vi "Main.vi"() -> ()   [LabVIEW 2017]
doc: "The myRIO Project template acquires acceleration data from the onboard accelerometer and displays the changes of acceleration values in a waveform chart."
uses:
  <vilib>/FPGAPlugInAG/myRIO-1900/niLvFpga_Open_myRIO-1900.vi
  <vilib>/rvi/interface/common/dynamic/niFpgaDynamicAddResources.vi
  <vilib>/Utility/error.llb/Error Cluster From Error Code.vi
  <vilib>/rvi/errors/niLvFpgaAdjustHostInterfaceError.vi
  <vilib>/FPGAPlugInAG/Dynamic/niLvFpga_Close_Dynamic.vi
  <vilib>/rvi/interface/nirviOpenFPGA/nirviOpenFPGA.xnode
  FPGA Bitfiles/BadassLoader_FPGATarget_DCMotorControlle_4dRX-8eX8o0.lvbitx
  <vilib>/rvi/interface/nirviReadWriteControl/nirviReadWriteControl.xnode
  <vilib>/rvi/interface/nirviCloseFPGA/nirviCloseFPGA.xnode
  <vilib>/rvi/interface/Simulation/niFpgaSimulationCallBeginRW.vi
  NiFpgaLv.dll
panel:
  out "Numeric Control":i32
  out "Servo 6":u32
  out "Servo 5":u32
  out "DCmotor_1_ccw vel":i32
  out "DCmotor_0_ccw vel":i32
  out "Speed":dbl(knob) scale=0.0..50.0
  out "Gear":u32(knob) scale=0.0..4.0
  out "Paused":bool
  out "Grab":bool
  in  "Stop":bool
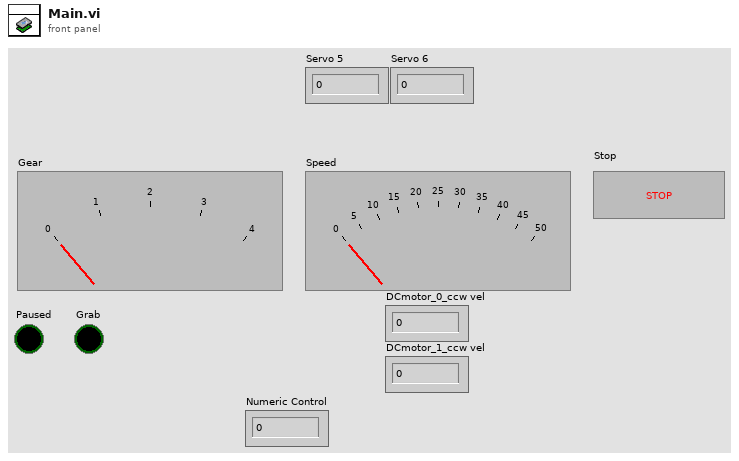
[diagram p1: front panel]
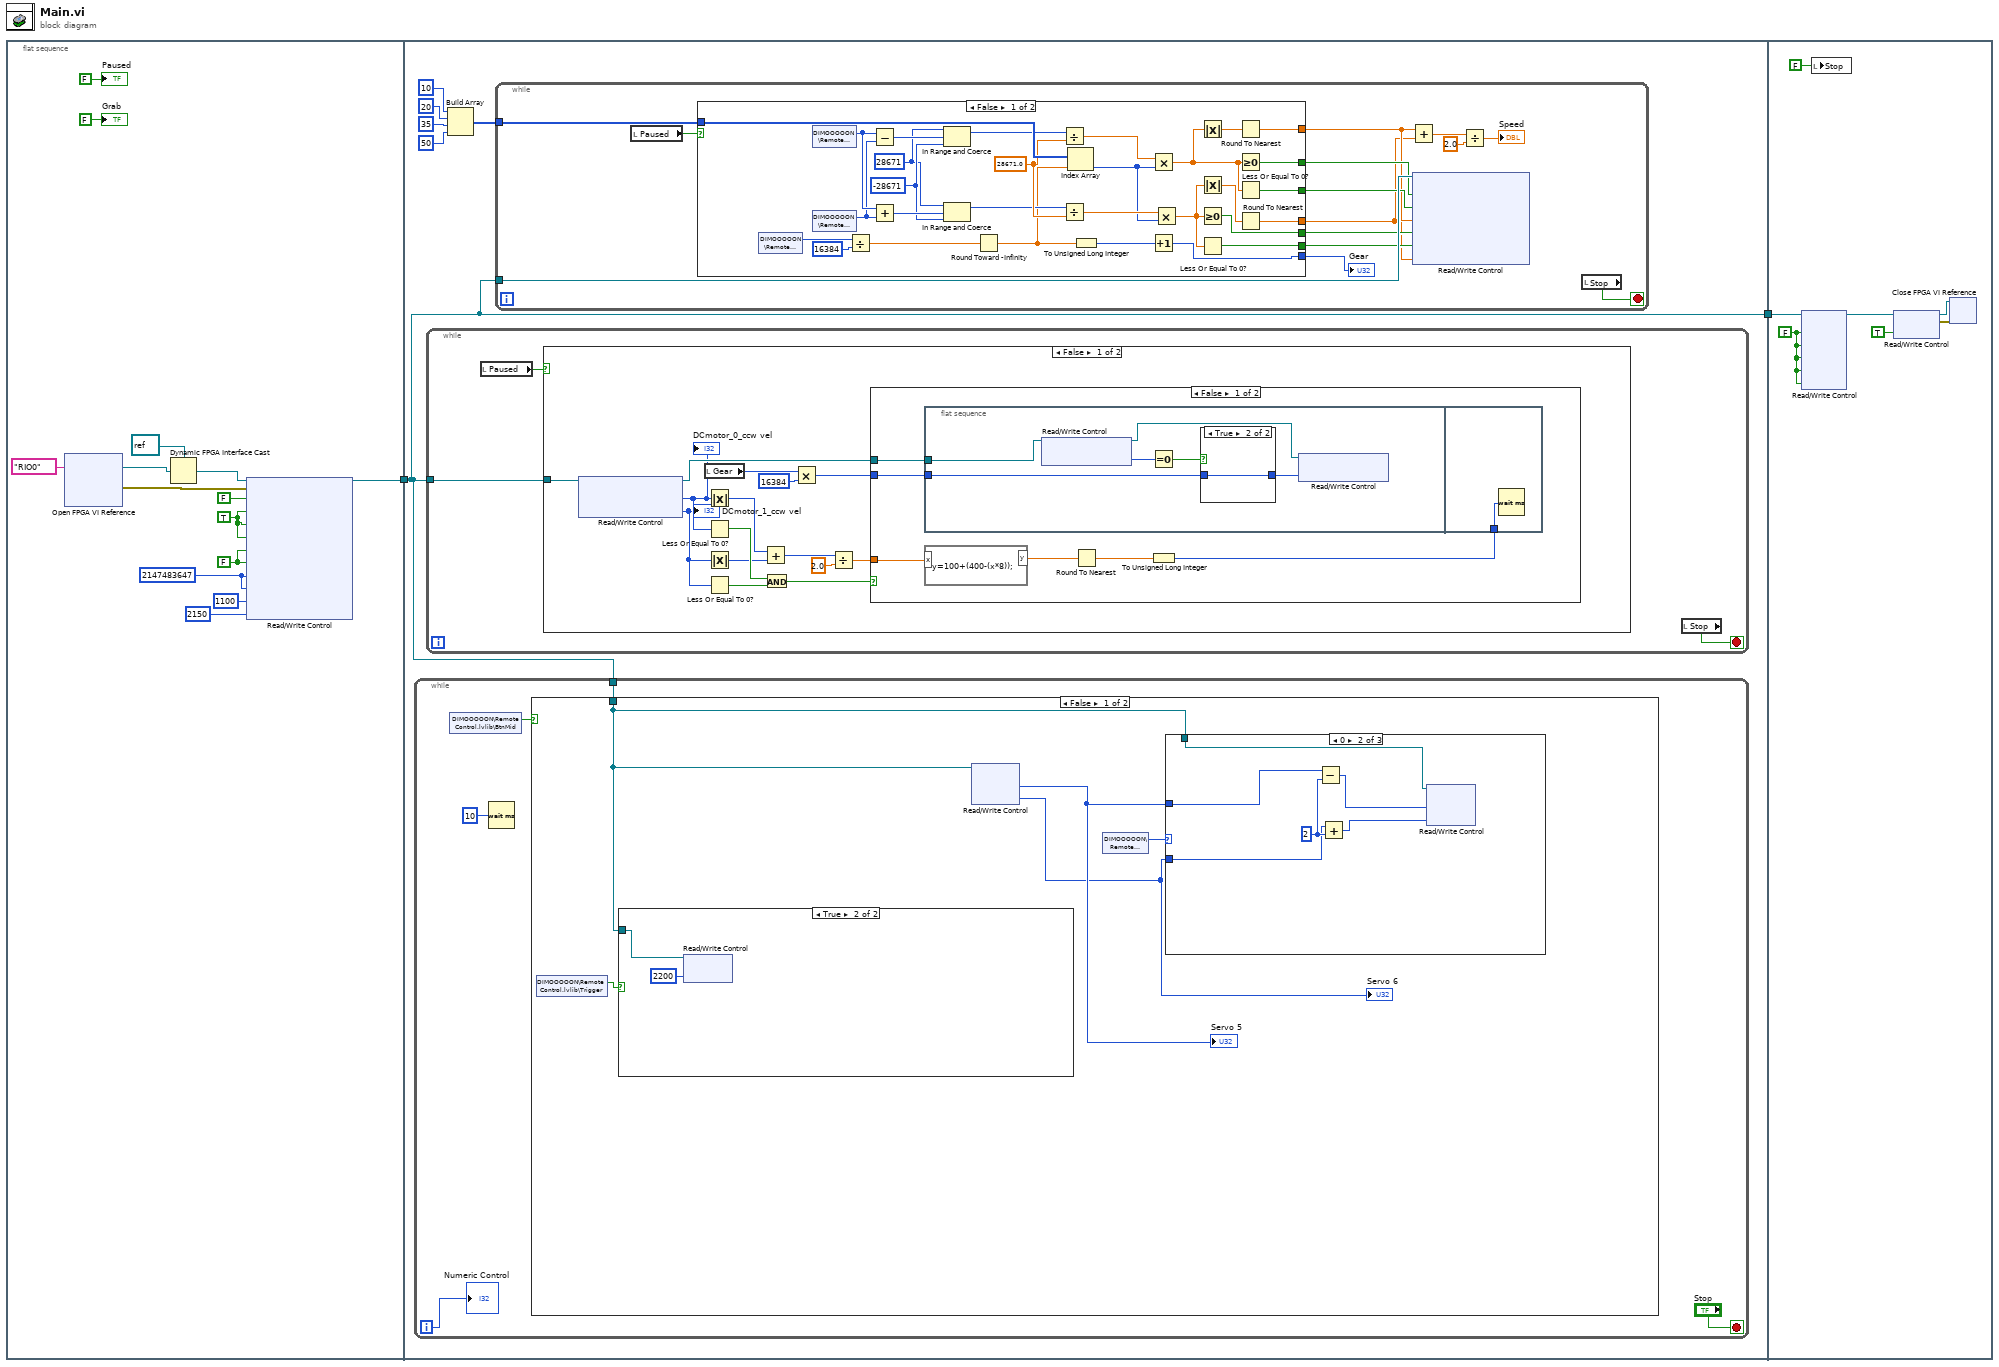
[diagram p0: block diagram]
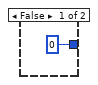
[diagram p2: hidden frame]
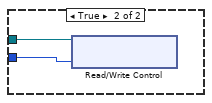
[diagram p3: hidden frame]
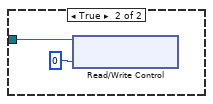
[diagram p4: hidden frame]
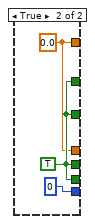
[diagram p5: hidden frame]
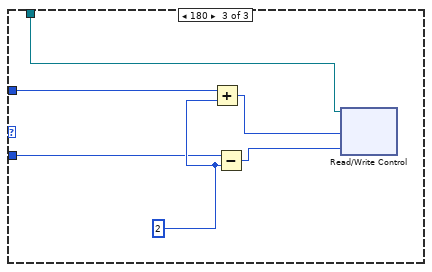
[diagram p7: hidden frame]
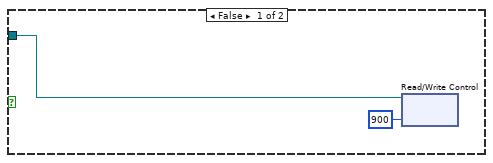
[diagram p8: hidden frame]
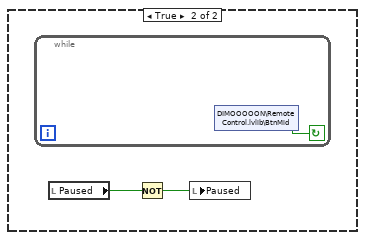
[diagram p9: hidden frame]
diagram:
  n1 = flat-sequence {
    tunnel: [w14] -> w1
    tunnel: [w17] -> w2
    tunnel: w1 -> [w17]
    tunnel: w2 -> [w138]
    frame #0 {
      w11 = FALSE
      w7 = TRUE ("S 4")
      w6 = 2147483647 ("DCmotor_1_enc trgt")
      n2 = xnode "Open FPGA VI Reference"("resource name"=tag "RIO0") -> ("FPGA VI Reference Out"=w9:refnum<k20>, "error out"=w10:errorcluster)  [unwired: 1 in]
      n3 = Dynamic FPGA Interface Cast(Session In=refnum<k20> refnum ("FPGA Interface"), Type=w9) -> (Session Out=w16:refnum<k20>)
      n4 = xnode "Read/Write Control"("FPGA VI Reference In"=w16, "error in"=w10, "invert pulse (F)"=FALSE, "S 4"=w7, "S 5"=w7, "S 6"=w7, "M0_finished"=w11, "M1_finished"=w11, "DCmotor_0_enc trgt"=w6, "DCmotor_1_enc trgt"=w6, "Servo 5"=u32 1100, "Servo 6"=u32 2150) -> ("FPGA VI Reference Out"=w14:refnum<k20>)  [unwired: 1 out]
      "Grab" <- FALSE
      "Paused" <- FALSE
    }
    frame #1 {
      n5 = while {
        tunnel: w17 -> [w107]
        i -> [w106]
        stop <- "Stop" stop-if-true
        n6 = shared-variable "DIMOOOOON\\Remote Control.lvlib\\BtnMid"() -> (w108:bool)  [unwired: 1 in, 1 out]
        n7 = Wait (ms)(milliseconds to wait=u32 10) -> ()  [unwired: 1 out]
        n8 = case shown="False" w108 {
          tunnel: w107 -> [w111 _]
          frame False {
            n9 = shared-variable "DIMOOOOON\\Remote Control.lvlib\\Trigger"() -> (w115:bool)  [unwired: 1 in, 1 out]
            n10 = case shown="True" w115 {
              tunnel: w111 -> [w128 w130]
              frame False {
                n11 = xnode "Read/Write Control"("FPGA VI Reference In"=w128, "Servo 4"=u32 900) -> ()  [unwired: 1 in, 2 out]
              }
              frame True {
                n12 = xnode "Read/Write Control"("FPGA VI Reference In"=w130, "Servo 4"=u32 2200) -> ()  [unwired: 1 in, 2 out]
              }
            }
            n13 = xnode "Read/Write Control"("FPGA VI Reference In"=w111) -> ("Servo 5"=w113:u32, "Servo 6"=w112:u32)  [unwired: 1 in, 2 out]
            "Servo 6" <- w112
            "Servo 5" <- w113
            n14 = shared-variable "DIMOOOOON\\Remote Control.lvlib\\LJ"() -> (w114:i16)  [unwired: 1 in, 1 out]
            n15 = case shown="0" w114 {
              tunnel: w111 -> [_ w121 w125]
              tunnel: w113 -> [_ w117 w123]
              tunnel: w112 -> [_ w116 w122]
              frame -1, Default {
              }
              frame 0 {
                w118 = u32 2 ("y")
                n16 = Subtract(x=w117, y=w118) -> (x-y=w120:u32)
                n17 = Add(x=w116, y=w118) -> (x+y=w119:u32)
                n18 = xnode "Read/Write Control"("FPGA VI Reference In"=w121, "Servo 5"=w120, "Servo 6"=w119) -> ()  [unwired: 1 in, 2 out]
              }
              frame 180 {
                w124 = u32 2 ("y")
                n19 = Add(x=w123, y=w124) -> (x+y=w127:u32)
                n20 = Subtract(x=w122, y=w124) -> (x-y=w126:u32)
                n21 = xnode "Read/Write Control"("FPGA VI Reference In"=w125, "Servo 5"=w127, "Servo 6"=w126) -> ()  [unwired: 1 in, 2 out]
              }
            }
          }
          frame True {
            n22 = while {
              stop <- w134 continue-if-true
              n23 = shared-variable "DIMOOOOON\\Remote Control.lvlib\\BtnMid"() -> (w134:bool)  [unwired: 1 in, 1 out]
            }
            n24 = local read "Paused"() -> (w133:bool)
            n25 = Not(x=w133) -> (.not. x?=w132:bool)
            n26 = local write "Paused"(w132) -> ()
          }
        }
        "Numeric Control" <- w106
      }
      n27 = while {
        tunnel: w17 -> [w23]
        stop <- w25 stop-if-true
        n28 = local read "Paused"() -> (w24:bool)
        n29 = case shown="False" w24 {
          tunnel: w23 -> [w37 w59]
          frame False {
            n30 = xnode "Read/Write Control"("FPGA VI Reference In"=w37) -> ("FPGA VI Reference Out"=w33:refnum<k20>, "DCmotor_0_ccw vel"=w32:i32, "DCmotor_1_ccw vel"=w31:i32)  [unwired: 1 in, 1 out]
            "DCmotor_0_ccw vel" <- w32
            "DCmotor_1_ccw vel" <- w31
            n31 = local read "Gear"() -> (w35:u32)
            n32 = Absolute Value(x=w32) -> (abs(x)=w28:i32)
            n33 = Less Or Equal To 0?(x=w32) -> (x <= 0?=w40:bool)
            n34 = Absolute Value(x=w31) -> (abs(x)=w27:i32)
            n35 = Less Or Equal To 0?(x=w31) -> (x <= 0?=w39:bool)
            n36 = Add(x=w28, y=w27) -> (x+y=w30:i32)
            n37 = And(x=w40, y=w39) -> (x .and. y?=w38:bool)
            n38 = Multiply(x=w35, y=u32 16384) -> (x*y=w36:u32)
            n39 = Divide(x=w30, y=2.0) -> (x/y=w26:dbl)
            n40 = case shown="False" w38 {
              tunnel: w33 -> [w46 w57]
              tunnel: w36 -> [w45 w56]
              tunnel: w26 -> [w42 _]
              frame False {
                n41 = flat-sequence {
                  tunnel: w46 -> [w52]
                  tunnel: w45 -> [w47]
                  tunnel: w43 -> [w55]
                  frame #0 {
                    n42 = xnode "Read/Write Control"("FPGA VI Reference In"=w52) -> ("FPGA VI Reference Out"=w50:refnum<k20>, "Overdrive Power"=w49:u32)  [unwired: 1 in, 1 out]
                    n43 = Equal To 0?(x=w49) -> (x = 0?=w48:bool)
                    n44 = case shown="True" w48 {
                      tunnel: [u32 0 w54] -> w51
                      tunnel: w47 -> [_ w54]
                      frame False {
                      }
                      frame True {
                      }
                    }
                    n45 = xnode "Read/Write Control"("FPGA VI Reference In"=w50, "Overdrive Power"=w51) -> ()  [unwired: 1 in, 2 out]
                  }
                  frame #1 {
                    n46 = Wait (ms)(milliseconds to wait=w55) -> ()  [unwired: 1 out]
                  }
                }
                n47 = formula code="y=100+(400-(x*8));"("x"=w42) -> ("y"=w41:dbl)
                n48 = Round To Nearest(number=w41) -> (nearest integer value=w44:dbl)
                n49 = To Unsigned Long Integer(number=w44) -> (unsigned 32bit integer=w43:u32)
              }
              frame True {
                n50 = xnode "Read/Write Control"("FPGA VI Reference In"=w57, "Overdrive Power"=w56) -> ()  [unwired: 1 in, 2 out]
              }
            }
          }
          frame True {
            n51 = xnode "Read/Write Control"("FPGA VI Reference In"=w59, "Overdrive Power"=u32 0) -> ()  [unwired: 1 in, 2 out]
          }
        }
        n52 = local read "Stop"() -> (w25:bool)
      }
      n53 = Build Array(i16 10 ("element"), i16 20 ("element"), i16 35 ("element"), i16 50 ("element")) -> (w18:i16[])
      n54 = while {
        tunnel: w17 -> [w72]
        tunnel: w18 -> [w66]
        stop <- w73 stop-if-true
        n55 = local read "Paused"() -> (w67:bool)
        n56 = case shown="False" w67 {
          tunnel: [w84 w105] -> w71
          tunnel: [w83 w105] -> w70
          tunnel: [w82 w105] -> w69
          tunnel: [w81 w105] -> w68
          tunnel: [w75 w104] -> w61
          tunnel: [w74 w104] -> w60
          tunnel: w66 -> [w102 _]
          tunnel: [w76 u32 0] -> w65
          frame False {
            w90 = -28671 ("element")
            w89 = 28671 ("element")
            w96 = 28671.0
            n57 = shared-variable "DIMOOOOON\\Remote Control.lvlib\\Z"() -> (w101:u32)  [unwired: 1 in, 1 out]
            n58 = shared-variable "DIMOOOOON\\Remote Control.lvlib\\Y"() -> (w95:i32)  [unwired: 1 in, 1 out]
            n59 = shared-variable "DIMOOOOON\\Remote Control.lvlib\\X"() -> (w94:i32)  [unwired: 1 in, 1 out]
            n60 = Divide(x=w101, y=16384) -> (x/y=w100:dbl)
            n61 = Subtract(x=w95, y=w94) -> (x-y=w93:i32)
            n62 = Add(x=w95, y=w94) -> (x+y=w92:i32)
            n63 = In Range and Coerce(upper limit=w89, x=w93, lower limit=w90) -> (coerced(x)=w88:i32)  [unwired: 1 out]
            n64 = In Range and Coerce(upper limit=w89, x=w92, lower limit=w90) -> (coerced(x)=w87:i32)  [unwired: 1 out]
            n65 = Round Toward -Infinity(1:w100) -> (0:w77:dbl)
            n66 = Divide(x=w88, y=w96) -> (x/y=w98:dbl)
            n67 = Divide(x=w87, y=w96) -> (x/y=w97:dbl)
            n68 = Index Array(array=w102, index=w77) -> (element=w91:i16)
            n69 = To Unsigned Long Integer(number=w77) -> (unsigned 32bit integer=w78:u32)
            n70 = Multiply(x=w98, y=w91) -> (x*y=w80:dbl)
            n71 = Increment(x=w78) -> (x+1=w76:u32)
            n72 = Multiply(x=w97, y=w91) -> (x*y=w79:dbl)
            n73 = Absolute Value(x=w80) -> (abs(x)=w86:dbl)
            n74 = Absolute Value(x=w79) -> (abs(x)=w85:dbl)
            n75 = Greater Or Equal To 0?(x=w79) -> (x >= 0?=w82:bool)
            n76 = Less Or Equal To 0?(x=w79) -> (x <= 0?=w81:bool)
            n77 = Round To Nearest(number=w86) -> (nearest integer value=w75:dbl)
            n78 = Greater Or Equal To 0?(x=w80) -> (x >= 0?=w84:bool)
            n79 = Less Or Equal To 0?(x=w80) -> (x <= 0?=w83:bool)
            n80 = Round To Nearest(number=w85) -> (nearest integer value=w74:dbl)
          }
          frame True {
            w104 = 0.0
            w105 = TRUE
          }
        }
        "Gear" <- w65
        n81 = Add(x=w61, y=w60) -> (x+y=w64:dbl)
        n82 = xnode "Read/Write Control"("FPGA VI Reference In"=w72, "DCmotor_0_A"=w71, "DCmotor_0_B"=w70, "DCmotor_0_ccw vel sp"=w61, "DCmotor_1_A"=w69, "DCmotor_1_B"=w68, "DCmotor_1_ccw vel sp"=w60) -> ()  [unwired: 1 in, 2 out]
        n83 = Divide(x=w64, y=2.0) -> (x/y=→"Speed":dbl)
        n84 = local read "Stop"() -> (w73:bool)
      }
    }
    frame #2 {
      w135 = FALSE
      n85 = xnode "Read/Write Control"("FPGA VI Reference In"=w138, "M2_A"=w135, "M2_B"=w135, "S 4"=w135, "S 6"=w135, "S 5"=w135) -> ("FPGA VI Reference Out"=w137:refnum<k20>)  [unwired: 1 in, 1 out]
      n86 = local write "Stop"(FALSE ("Stop")) -> ()
      n87 = xnode "Read/Write Control"("FPGA VI Reference In"=w137, "stop"=TRUE) -> ("FPGA VI Reference Out"=w140:refnum<k20>, "error out"=w141:errorcluster)  [unwired: 1 in]
      n88 = xnode "Close FPGA VI Reference"("FPGA VI Reference In"=w140, "error in"=w141) -> ()  [unwired: 1 out]
    }
  }
